vi "User Dynamic (multiple).vi"(7 "User.lvclass":refnum<class "User.lvclass">, 8 "error in (no error)":errorcluster, 11 "XY-data":cluster{"X-array":dbl[], "Y-array":dbl[]}[](array[cluster]) {"Y-array" format="%.2p"; "X-array" format="%.2p"}) -> (0 "error out":errorcluster, 3 "XY-data out":cluster{"X-array":dbl[], "Y-array":dbl[]}[](array[cluster]) {"Y-array" format="%.2p"; "X-array" format="%.2p"}, 5 "User.lvclass out":refnum<class "User.lvclass">)   [LabVIEW 2019, in "User.lvclass"]
uses:
  User.lvclass
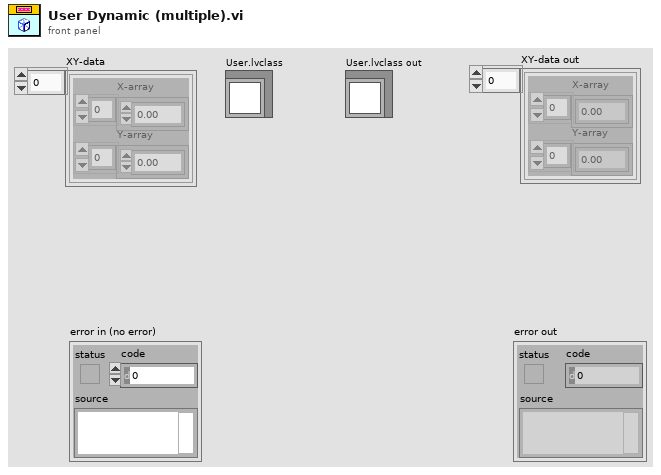
[diagram p1: front panel]
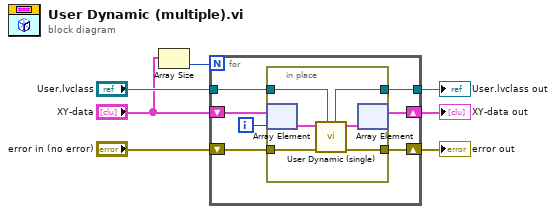
[diagram p0: block diagram]
diagram:
  n1 = Array Size(array="XY-data") -> (size(s)=w4:i32)
  n2 = for {
    N: w4 -> [_]
    tunnel: "User.lvclass" -> [w14]
    shift-right: [w13] -> w2
    shift-left: "XY-data" -> [w9]
    shift-right: [w10] -> w6
    shift-left: "error in (no error)" -> [w11]
    tunnel: [w8] -> w1
    i -> [w12]
    n3 = in-place {
      in-place-border: w14 -> [w16]
      in-place-border: w11 -> [w18]
      in-place-border: [w17] -> w10
      in-place-border: [w15] -> w8
      n4 = in-place-array #1(w9, w12) -> (w20:cluster{"X-array":dbl[], "Y-array":dbl[]})
      n5 = call-dynamic "User Dynamic (single).vi"("User.lvclass"=w16, "error in (no error)"=w18, "XY-data"=w20) -> ("error out"=w17:errorcluster, "XY-data out"=w19:cluster{"X-array":dbl[], "Y-array":dbl[]}, "User.lvclass out"=w15:refnum<class "User.lvclass">)  [unwired: 6 in]
      n6 = in-place-array #1(w19) -> (w13:cluster{"X-array":dbl[], "Y-array":dbl[]}[])  [unwired: 1 out]
    }
  }
  "error out" <- w6
  "XY-data out" <- w2
  "User.lvclass out" <- w1
